vi "ANAL Time date.vi"(8 "タイムスタンプ":timestamp, 11 "Before":string) -> (3 "Anal Time":string)   [LabVIEW 2018]
panel:
  out "数値 8":i32
  out "数値 7":i32
  out "H":i32
  out "M":i32
  out "S":i32
  out "x - y":i32
  out "結果 2":i32
  out "数値 6":i32
  out "数値 5":i32
  out "数値 4":i32
  out "部分文字列の後 2":string
  out "部分文字列の前 4":string
  out "部分文字列の前 3":string
  out "結果":i32
  out "数値 3":i32
  out "数値 2":i32
  out "数値":i32
  out "部分文字列の後":string
  out "部分文字列の前 2":string
  out "部分文字列の前":string
  out "after":string
  # "01:00:05:50"
  # "28:23:59:30"
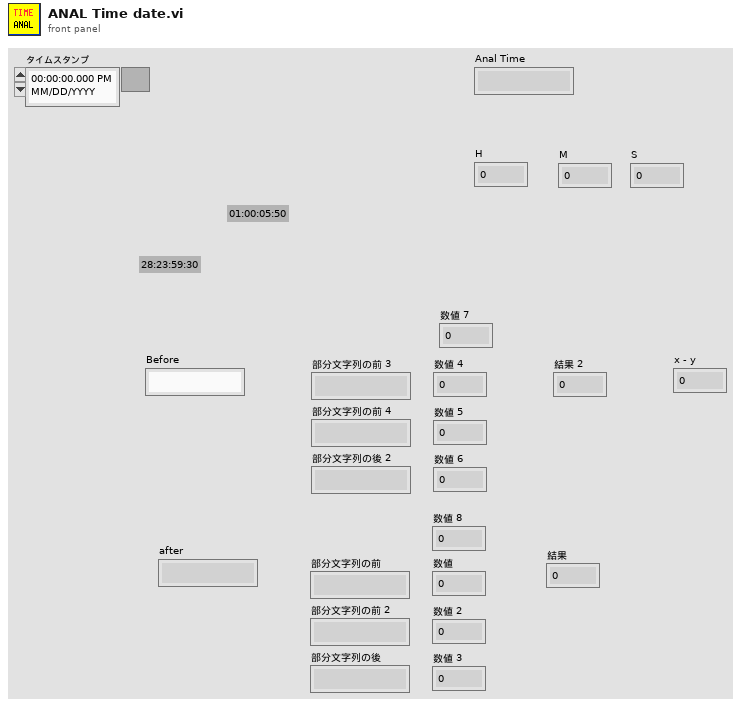
[diagram p1: front panel]
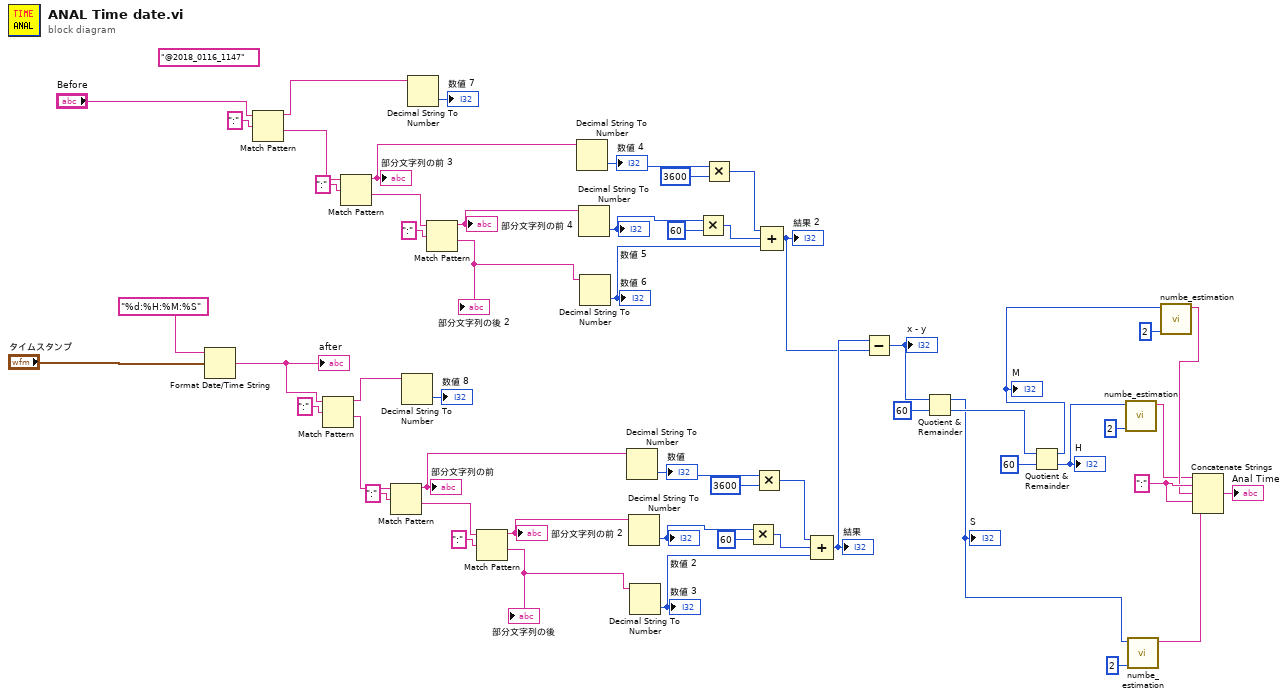
[diagram p0: block diagram]
diagram:
  (unwired) "@2018_0116_1147" ("Date")
  w22 = ":" ("文字列")
  n1 = Format Date/Time String(time format string (%c)="%d:%H:%M:%S" ("時間形式文字列（%c）"), seconds (now)="タイムスタンプ") -> (date/time string=w9:string)  [unwired: 1 in]
  "after" <- w9
  n2 = Match Pattern(string="Before", regular expression=":" ("検索文字列")) -> (before substring=w3:string, after substring=w5:string)  [unwired: 1 in, 2 out]
  n3 = Match Pattern(string=w9, regular expression=":" ("検索文字列")) -> (before substring=w1:string, after substring=w8:string)  [unwired: 1 in, 2 out]
  n4 = Match Pattern(string=w5, regular expression=":" ("検索文字列")) -> (before substring=w38:string, after substring=w39:string)  [unwired: 1 in, 2 out]
  "部分文字列の前 3" <- w38
  n5 = Match Pattern(string=w8, regular expression=":" ("検索文字列")) -> (before substring=w51:string, after substring=w52:string)  [unwired: 1 in, 2 out]
  "部分文字列の前" <- w51
  n6 = Decimal String To Number(string=w1) -> (number=→"数値 8":i32)  [unwired: 2 in, 1 out]
  n7 = Decimal String To Number(string=w3) -> (number=→"数値 7":i32)  [unwired: 2 in, 1 out]
  n8 = Match Pattern(string=w39, regular expression=":" ("検索文字列")) -> (before substring=w37:string, after substring=w36:string)  [unwired: 1 in, 2 out]
  "部分文字列の前 4" <- w37
  "部分文字列の後 2" <- w36
  n9 = Match Pattern(string=w52, regular expression=":" ("検索文字列")) -> (before substring=w50:string, after substring=w49:string)  [unwired: 1 in, 2 out]
  "部分文字列の前 2" <- w50
  "部分文字列の後" <- w49
  n10 = Decimal String To Number(string=w38) -> (number=w32:i32)  [unwired: 2 in, 1 out]
  "数値 4" <- w32
  n11 = Decimal String To Number(string=w37) -> (number=w35:i32)  [unwired: 2 in, 1 out]
  "数値 5" <- w35
  n12 = Decimal String To Number(string=w36) -> (number=w29:i32)  [unwired: 2 in, 1 out]
  "数値 6" <- w29
  n13 = Decimal String To Number(string=w51) -> (number=w45:i32)  [unwired: 2 in, 1 out]
  "数値" <- w45
  n14 = Decimal String To Number(string=w50) -> (number=w48:i32)  [unwired: 2 in, 1 out]
  "数値 2" <- w48
  n15 = Decimal String To Number(string=w49) -> (number=w42:i32)  [unwired: 2 in, 1 out]
  "数値 3" <- w42
  n16 = Multiply(x=w35, y=60) -> (x*y=w30:i32)
  n17 = Multiply(x=w32, y=3600) -> (x*y=w31:i32)
  n18 = Multiply(x=w48, y=60) -> (x*y=w43:i32)
  n19 = Multiply(x=w45, y=3600) -> (x*y=w44:i32)
  n20 = Compound Arithmetic op=ADD(w31, w30, w29) -> (w27:i32)
  "結果 2" <- w27
  n21 = Compound Arithmetic op=ADD(w44, w43, w42) -> (w28:i32)
  "結果" <- w28
  n22 = Subtract(x=w28, y=w27) -> (x-y=w26:i32)
  "x - y" <- w26
  n23 = Quotient & Remainder(x=w26, y=60) -> (x-y*floor(x/y)=w17:i32, floor(x/y)=w23:i32)
  "S" <- w17
  n24 = Quotient & Remainder(x=w23, y=60) -> (x-y*floor(x/y)=w15:i32, floor(x/y)=w12:i32)
  "M" <- w15
  "H" <- w12
  n25 = call "numbe_estimation.vi"("桁数"=2, "数値"=w12) -> ("数値文字列"=w11:string)  [unwired: 9 in]
  n26 = call "numbe_estimation.vi"("桁数"=2, "数値"=w17) -> ("数値文字列"=w16:string)  [unwired: 9 in]
  n27 = call "numbe_estimation.vi"("桁数"=2, "数値"=w15) -> ("数値文字列"=w14:string)  [unwired: 9 in]
  n28 = Concatenate Strings(w11, w22, w14, w22, w16) -> (→"Anal Time":string)
